vi "Test_AI.vi"() -> ()   [LabVIEW 2026]
doc: "AI_Calculate_Move 테스트."
panel:
  out "error out":errorcluster
  out "Valid":bool
  out "Score":dbl
  out "Col":i32
  out "Row":i32
  in  "Renju":bool=TRUE
  in  "Difficulty":enum8{"Easy", "Normal", "Hard", "Master"}(ring)=enum."Normal"
  in  "AI Stone":i32=2
  in  "Stones":i32[](array[numeric])=[1, 1, 1, 1]
  in  "Cols":i32[](array[numeric])=[3, 4, 5, 6]
  in  "Rows":i32[](array[numeric])=[7, 7, 7, 7]
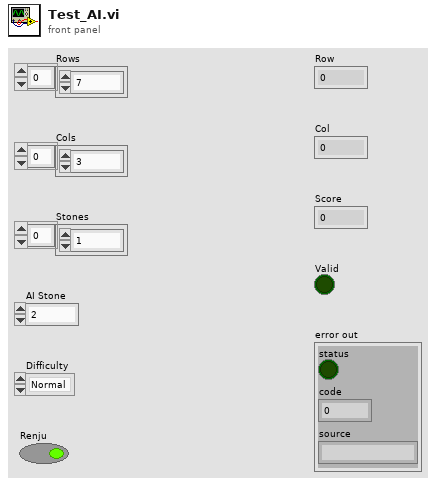
[diagram p1: front panel]
types:
  T1 = cluster{"Row":i32, "Col":i32, "Stone":enum8{"Empty", "Black", "White"}}
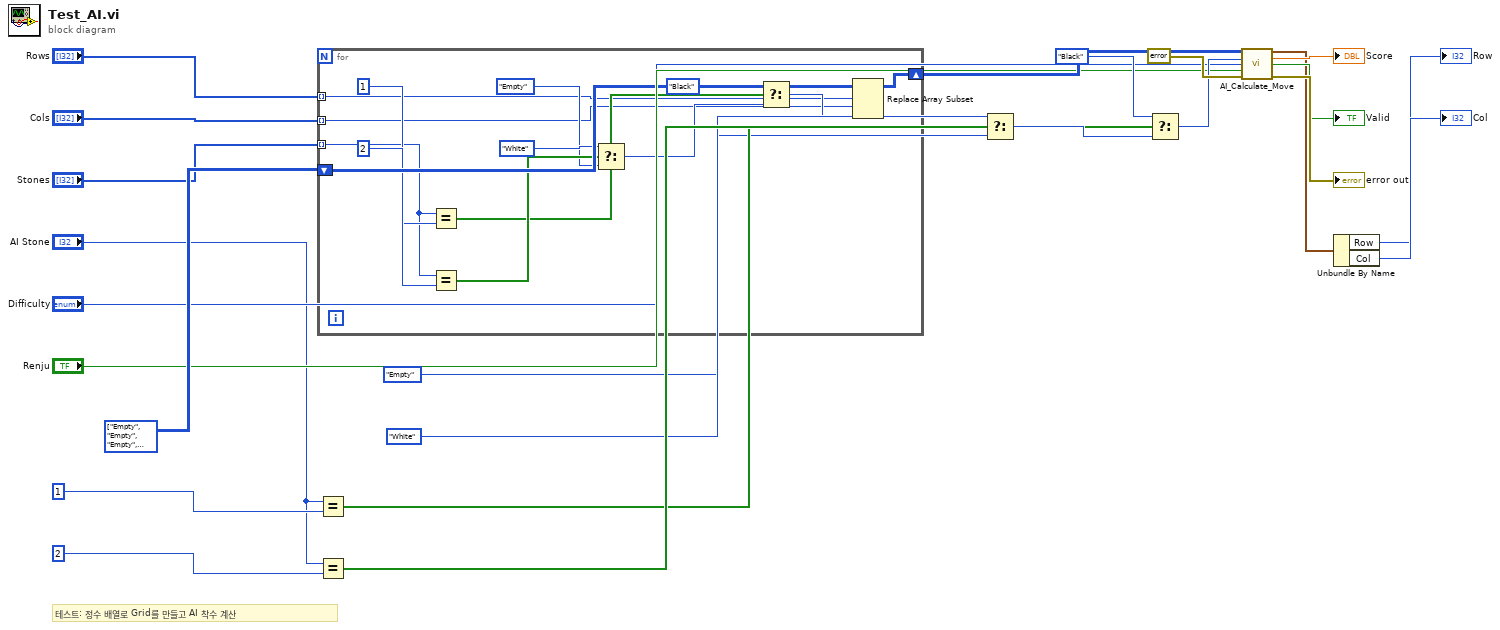
[diagram p0: block diagram]
diagram:
  w7 = enum8{"Empty", "Black", "White"}[][] [[enum."Empty", enum."Empty", enum."Empty", enum."Empty", enum."Empty", enum."Empty", enum."Empty", enum."Empty", enum."Empty", enum."Empty", enum."Empty", enum."Empty", enum."Empty", enum."Empty", enum."Empty"], [enum."Empty", enum."Empty", enum."Empty", enum."Empty", enum."Empty", enum."Empty", enum."Empty", enum."Empty", enum."Empty", enum."Empty", enum."Empty", enum."Empty", enum."Empty", enum."Empty", enum."Empty"], [enum."Empty", enum."Empty", enum."Empty", enum."Empty", enum."Empty", enum."Empty", enum."Empty", enum."Empty", enum."Empty", enum."Empty", enum."Empty", enum."Empty", enum."Empty", enum."Empty", enum."Empty"], [enum."Empty", enum."Empty", enum."Empty", enum."Empty", enum."Empty", enum."Empty", enum."Empty", enum."Empty", enum."Empty", enum."Empty", enum."Empty", enum."Empty", enum."Empty", enum."Empty", enum."Empty"], [enum."Empty", enum."Empty", enum."Empty", enum."Empty", enum."Empty", enum."Empty", enum."Empty", enum."Empty", enum."Empty", enum."Empty", enum."Empty", enum."Empty", enum."Empty", enum."Empty", enum."Empty"], [enum."Empty", enum."Empty", enum."Empty", enum."Empty", enum."Empty", enum."Empty", enum."Empty", enum."Empty", enum."Empty", enum."Empty", enum."Empty", enum."Empty", enum."Empty", enum."Empty", enum."Empty"], [enum."Empty", enum."Empty", enum."Empty", enum."Empty", enum."Empty", enum."Empty", enum."Empty", enum."Empty", enum."Empty", enum."Empty", enum."Empty", enum."Empty", enum."Empty", enum."Empty", enum."Empty"], [enum."Empty", enum."Empty", enum."Empty", enum."Empty", enum."Empty", enum."Empty", enum."Empty", enum."Empty", enum."Empty", enum."Empty", enum."Empty", enum."Empty", enum."Empty", enum."Empty", enum."Empty"], [enum."Empty", enum."Empty", enum."Empty", enum."Empty", enum."Empty", enum."Empty", enum."Empty", enum."Empty", enum."Empty", enum."Empty", enum."Empty", enum."Empty", enum."Empty", enum."Empty", enum."Empty"], [enum."Empty", enum."Empty", enum."Empty", enum."Empty", enum."Empty", enum."Empty", enum."Empty", enum."Empty", enum."Empty", enum."Empty", enum."Empty", enum."Empty", enum."Empty", enum."Empty", enum."Empty"], [enum."Empty", enum."Empty", enum."Empty", enum."Empty", enum."Empty", enum."Empty", enum."Empty", enum."Empty", enum."Empty", enum."Empty", enum."Empty", enum."Empty", enum."Empty", enum."Empty", enum."Empty"], [enum."Empty", enum."Empty", enum."Empty", enum."Empty", enum."Empty", enum."Empty", enum."Empty", enum."Empty", enum."Empty", enum."Empty", enum."Empty", enum."Empty", enum."Empty", enum."Empty", enum."Empty"], [enum."Empty", enum."Empty", enum."Empty", enum."Empty", enum."Empty", enum."Empty", enum."Empty", enum."Empty", enum."Empty", enum."Empty", enum."Empty", enum."Empty", enum."Empty", enum."Empty", enum."Empty"], [enum."Empty", enum."Empty", enum."Empty", enum."Empty", enum."Empty", enum."Empty", enum."Empty", enum."Empty", enum."Empty", enum."Empty", enum."Empty", enum."Empty", enum."Empty", enum."Empty", enum."Empty"], [enum."Empty", enum."Empty", enum."Empty", enum."Empty", enum."Empty", enum."Empty", enum."Empty", enum."Empty", enum."Empty", enum."Empty", enum."Empty", enum."Empty", enum."Empty", enum."Empty", enum."Empty"]] items=["Empty", "Black", "White"]
  # "테스트: 정수 배열로 Grid를 만들고 AI 착수 계산"
  n1 = for {
    tunnel: "Rows" -> [w25] mode=indexing
    tunnel: "Cols" -> [w26] mode=indexing
    tunnel: "Stones" -> [w27] mode=indexing
    shift-right: [w37] -> w8
    shift-left: w7 -> [w38]
    n2 = Equal?(x=w27, y=1) -> (x = y?=w32:bool[])
    n3 = Equal?(x=w27, y=2) -> (x = y?=w34:bool[])
    n4 = Select(t=enum8{"Empty", "Black", "White"}."White", s=w34, f=enum8{"Empty", "Black", "White"}."Empty") -> (s? t:f=w35:enum8{"Empty", "Black", "White"})
    n5 = Select(t=enum8{"Empty", "Black", "White"}."Black", s=w32, f=w35) -> (s? t:f=w36:enum8{"Empty", "Black", "White"})
    n6 = Replace Array Subset(array=w38, new element=w36, index (row)=w25, index (col)=w26) -> (w37:enum8{"Empty", "Black", "White"}[][])
  }
  n7 = Equal?(x="AI Stone", y=1) -> (x = y?=w13:bool[])
  n8 = Equal?(x="AI Stone", y=2) -> (x = y?=w15:bool[])
  n9 = Select(t=enum8{"Empty", "Black", "White"}."White", s=w15, f=enum8{"Empty", "Black", "White"}."Empty") -> (s? t:f=w16:enum8{"Empty", "Black", "White"})
  n10 = Select(t=enum8{"Empty", "Black", "White"}."Black", s=w13, f=w16) -> (s? t:f=w17:enum8{"Empty", "Black", "White"})
  n11 = call "AI_Calculate_Move.vi"("Grid"=w8, "AI Stone"=w17, "Difficulty"="Difficulty", "Renju"="Renju", "error in"=errorcluster {"status"=FALSE, "code"=0, "source"=""}) -> ("Move"=w19:T1, "Score"=→"Score":dbl, "Valid"=→"Valid":bool, "error out"=→"error out":errorcluster)  [unwired: 7 in]
  n12 = Unbundle By Name(w19) -> ("Row"=→"Row":i32, "Col"=→"Col":i32)
